vi "4Pi Dual DM - Mode Scan Engine.vi"() -> ()   [LabVIEW 2021]
uses:
  4Pi Dual DM - Controls/4Pi Dual DM - Mode Scan - Gaussian Initial Guesses.ctl
  4Pi Dual DM - Controls/4Pi Dual DM - Mode Scan - Metric Fit Type.ctl
  4Pi Dual DM - Controls/4Pi Dual DM - Mode Scan - Scan Settings.ctl
  4Pi Dual DM - Controls/4Pi Dual DM - Mode Scan - Metric.ctl
  4Pi Dual DM - Controls/4Pi Dual DM - Mode Scan - Threshold Mean Limits.ctl
  4Pi Dual DM - Controls/4Pi Dual DM - Mode Scan - Image Type.ctl
  4Pi Dual DM - Controls/4Pi Dual DM - Mode Scan - Blink Scan Settings.ctl
  4Pi Dual DM - Controls/4Pi Dual DM - Mode Scan - Blink Analysis Type.ctl
  <vilib>/vision/Image Controls.llb/IMAQ Image.ctl
  Hardware Configuration/Hardware Configuration Controls/Device Type.ctl
  Hardware Configuration/Hardware Configuration Controls/Device Function.ctl
  <vilib>/Utility/miscctls.llb/LVPointTypeDef.ctl
  4Pi Dual DM - Controls/4Pi Dual DM - Mode Scan - Last Used Data Type.ctl
  4Pi Dual DM - Controls/4Pi Dual DM - Mode Scan - Notifier Type.ctl
  4Pi Dual DM - Controls/4Pi Dual DM - Mode Scan - Scan Actions.ctl
  4Pi Dual DM - Controls/4Pi Dual DM - Standard Action.ctl
  4Pi Dual DM - Controls/4Pi Dual DM - Standard Counter Action.ctl
  <vilib>/Analysis/6fits.llb/Curve Fitting Criteria.ctl
  <vilib>/Analysis/baseanly.llb/Mean (DBL).vi
  <vilib>/Analysis/NI_AALBase.lvlib
  <vilib>/Analysis/NI_AALPro.lvlib
  <vilib>/gmath/NI_Gmath.lvlib
  <resource>/objmgr/IMAQImage.rc
panel:
  in  "Calling VI Ref":refnum<vi>
  in  "Main Tab":enum32{"Scan Modes", "Settings"}(tab)
  in  "Fit Data":bool
  in  "Apply":bool
  in  "Get Image":bool
  in  "Current Mode":i32(ring) items=["1", "2", "3", "4", "5", "6", "7", "8", "9", "10", "11", "12", "13", "14", "15", "16", "17", "18", "19", "20", "21", "22", "23", "24", "25", "26", "27", "28", "29", "30", "31", "32", "33", "34", "35", "36", "37", "38", "39", "40", "41", "42", "43", "44", "45", "46", "47", "48", "49", "50", "51", "52", "53", "54", "55", "56", "57", "58", "59", "60", "61", "62", "63", "64", "65", "66", "67", "68", "69", "70", "71", "72", "73", "74", "75", "76", "77", "78", "79", "80", "81", "82", "83", "84", "85", "86", "87", "88", "89", "90", "91", "92", "93", "94", "95", "96", "97", "98", "99", "100", "101", "102", "103", "104", "105", "106", "107", "108", "109", "110", "111", "112", "113", "114", "115", "116", "117", "118", "119", "120", "121", "122", "123", "124", "125", "126", "127", "128", "129", "130", "131", "132", "133", "134", "135", "136", "137", "138", "139", "140"]
  in  "Scan Mode":bool
  in  "Scan Next Mode":bool
  in  "Auto Scan Modes":bool
  out "Metric":cluster{dbl[], dbl[]}[](graph)
  out "AO Image Display":T1(plugin-control)
  in  "Gaussian Initial Guesses":T2={"Amplitude"=2500.0, "Center Position"=0.0, "Width (Sigma)"=200.0, "Offset"=500.0, "User Guesses"=TRUE}
  in  "DM Scan Settings":T3={"Frame Delay"=1, "Frame Accumulations"=2, "Number of Steps"=8, "Step Size (nm)"=0.5} {"Step Size (nm)" format="%.2f"}
  in  "Image Type":T4 items=["Full Image", "ROI", "Blinks"]
  in  "Image Selection":i32(ring) items=["Quad 01", "Quad 02", "Quad 03", "Quad 04"]
  in  "Metric":T5=1 items=["Max Intensity", "No Zero Mean", "Threshold Mean", "Mean"]
  in  "Metric Fit Type":T6 items=["Guassian", "Quadratic"]
  in  "Threshold Mean Limits":T7={"Upper Limit"=10000.0, "Lower Limit"=0.0}
  in  "Blink Scan Settings":T8={"Blink Analysis Type"=1, "Blink ROI Box Width"=0, "Blink Threshold"=0.0} {"Blink Analysis Type" items=["Mean Intensity", "2D Fit Intensity"]}
  in  "Exit":bool
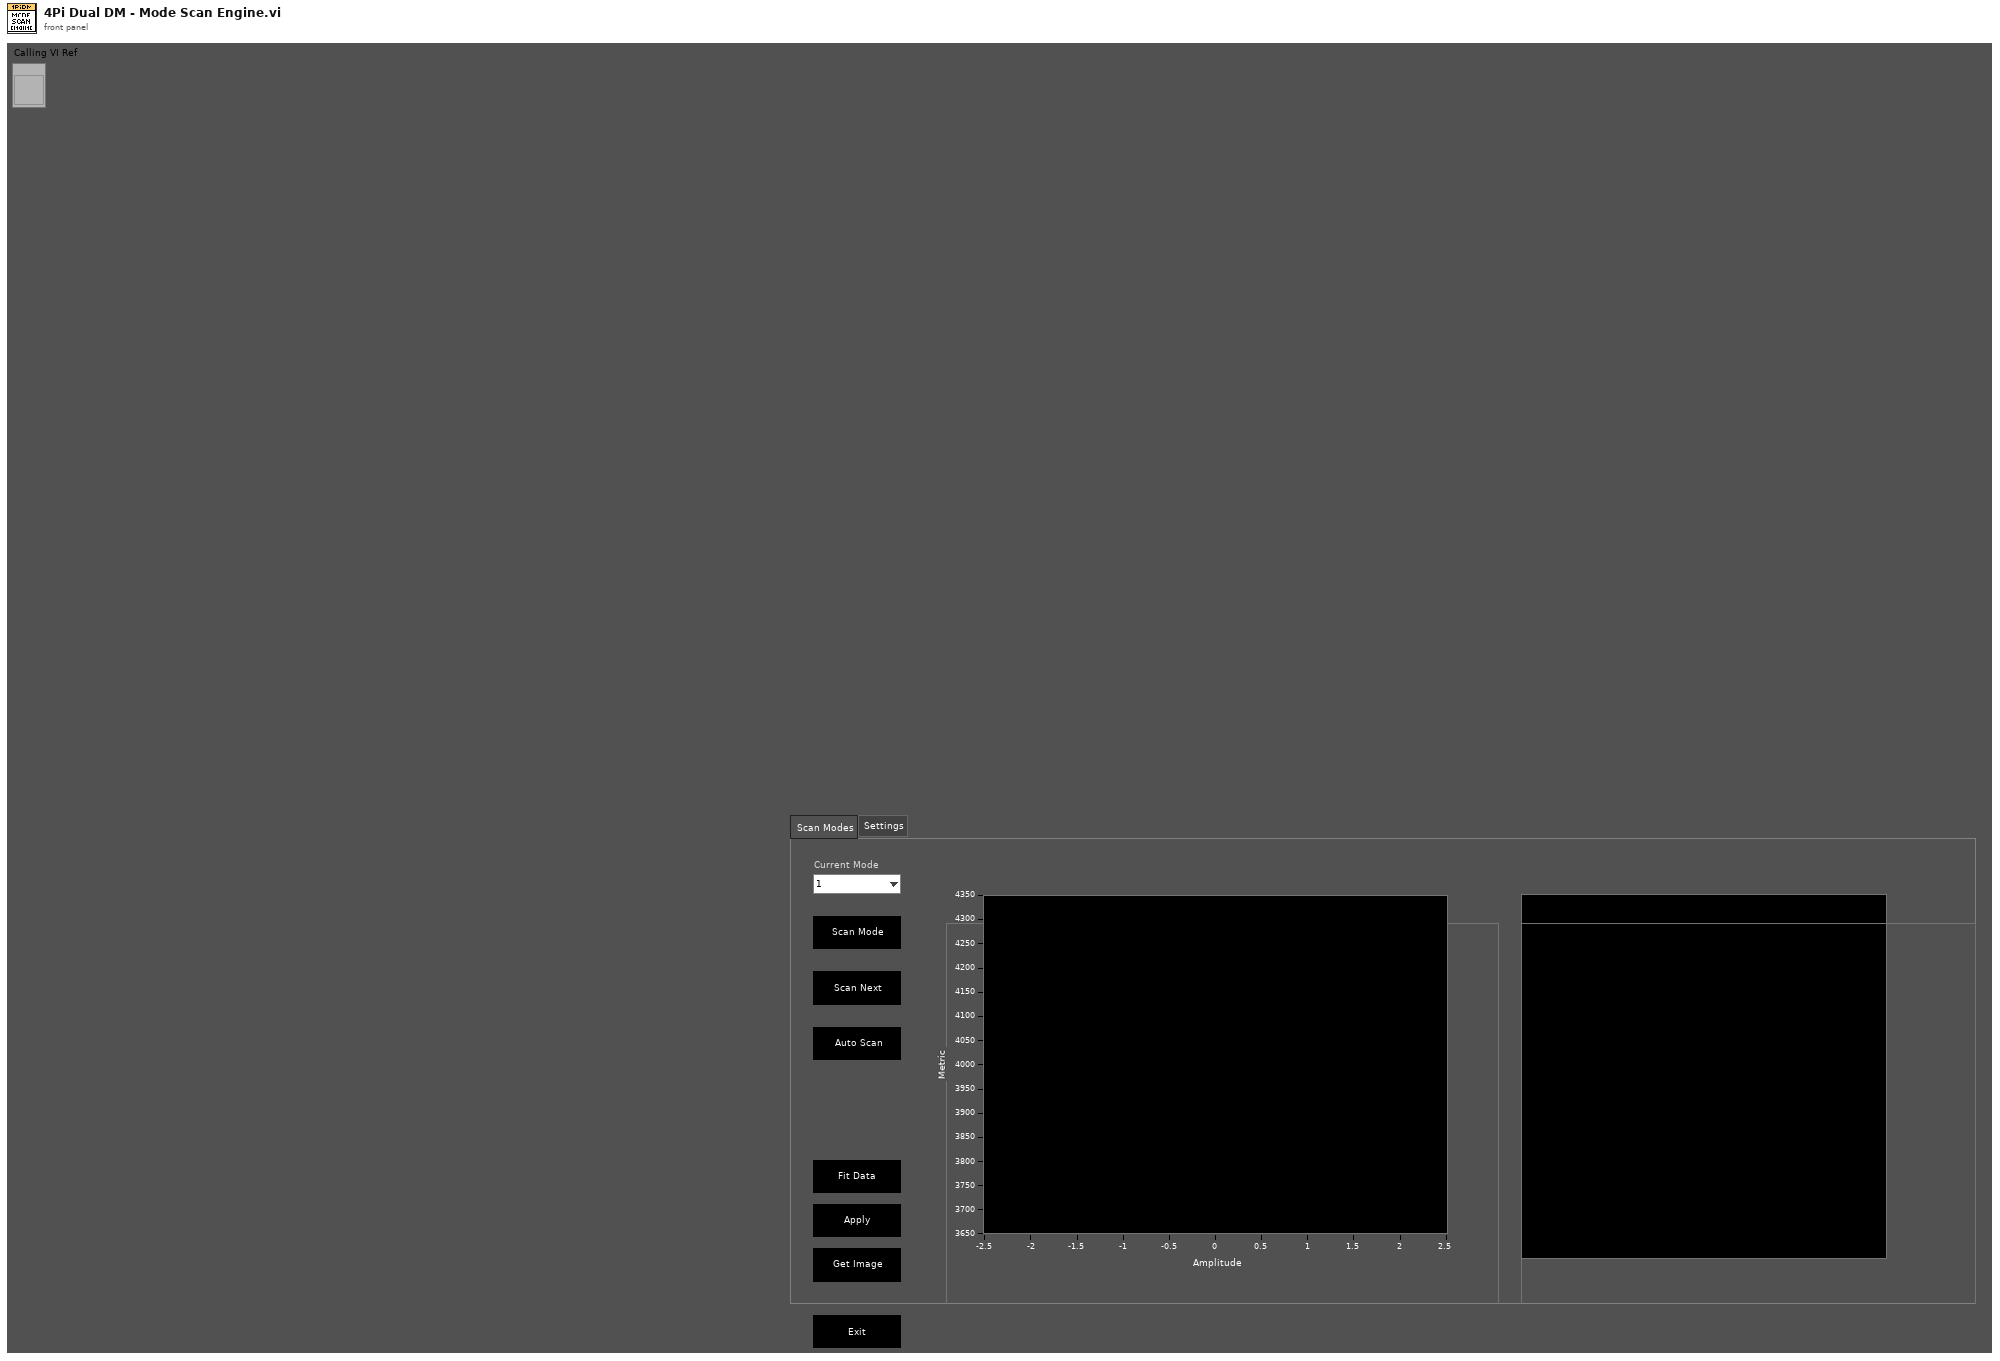
[diagram p1: front panel]
types:
  T1 = typedef "IMAQ Image.ctl" = refnum<image>
  T2 = typedef "4Pi Dual DM - Mode Scan - Gaussian Initial Guesses.ctl" = cluster{"Amplitude":dbl, "Center Position":dbl, "Width (Sigma)":dbl, "Offset":dbl, "User Guesses":bool}
  T3 = typedef "4Pi Dual DM - Mode Scan - Scan Settings.ctl" = cluster{"Frame Delay":u32, "Frame Accumulations":u16, "Number of Steps":u16, "Step Size (nm)":dbl}
  T4 = typedef "4Pi Dual DM - Mode Scan - Image Type.ctl" = u16
  T5 = typedef "4Pi Dual DM - Mode Scan - Metric.ctl" = u16
  T6 = typedef "4Pi Dual DM - Mode Scan - Metric Fit Type.ctl" = u16
  T7 = typedef "4Pi Dual DM - Mode Scan - Threshold Mean Limits.ctl" = cluster{"Upper Limit":dbl, "Lower Limit":dbl}
  T8 = typedef "4Pi Dual DM - Mode Scan - Blink Scan Settings.ctl" = cluster{"Blink Analysis Type":T9, "Blink ROI Box Width":u8, "Blink Threshold":sgl}
  T9 = typedef "4Pi Dual DM - Mode Scan - Blink Analysis Type.ctl" = u16
  T10 = typedef "Image Type" = u32
  T11 = enum8{"Enabled", "Disabled", "Disabled and Grayed Out"}
  T12 = typedef "4Pi Dual DM - Mode Scan - Scan Actions.ctl" = enum16{"Scan Mode", "Fit Data", "Scan Next Mode", "Update Mode Amount", "Get Image", "Compute Metric", "Update Counter", "Apply Correction", "Exit", "Quit"}
  T13 = typedef "4Pi Dual DM - Mode Scan - Notifier Type.ctl" = cluster{"Action":T12, "Image Ref":T1, "Image Type":T4, "Fit Type":T6, "Metric":T5, "Scan Running?":bool, "DM Scan Settings":T3, "Threshold Mean Limits":T7, "Gaussian Initial Guesses":T2, "Blink Scan Settings":T8}
  T14 = typedef "4Pi Dual DM - Mode Scan - Last Used Data Type.ctl" = cluster{"Image Ref Index":i32, "Image Type":T4, "Fit Type":T6, "Metric":T5, "DM Scan Settings":T3, "Threshold Mean Limits":T7, "Gaussian Initial Guesses":T2, "Blink Scan Settings":T8}
  T15 = enum16{"Always On", "Always Off", "Off While Running"}
  T16 = typedef "LVPointTypeDef.ctl" = cluster{"Horizontal":i16, "Vertical":i16}
  T17 = typedef "Device Function.ctl" = enum16{"Primary", "Secondary", "Overview", "Wide Field Drift Correction", "642 nm Excitation", "560 nm Excitation", "940 nm Excitation", "546 nm Excitation", "488 nm Excitation", "405 nm Excitation", "Objective Drift Correction", "4Pi Focus Lock", "4Pi Objective Lock", "Objective XY", "Objective Z", "Sample XY", "Sample Coarse Z", "Sample Z", "4Pi Lower", "4Pi Upper", "Em Small", "Em Large", "Ex Small", "Ex Large", "Mojo", "Adj Cavity", "Line Scanning", "Alert"}
  T18 = typedef "Device Type.ctl" = enum16{"AOTF", "Camera", "Deformable Mirror", "Laser", "Flip Mirror", "Shutter", "Stage", "Waveform", "FPGA", "Email"}
  T19 = typedef "LVRectTypeDef.ctl" = cluster{"Left":i16, "Top":i16, "Right":i16, "Bottom":i16}
  T20 = typedef "LVBoundsTypeDef.ctl" = cluster{"Width":u32, "Height":u32}
  T21 = typedef "4Pi Dual DM - Standard Action.ctl" = enum16{"Read", "Write"}
  T22 = typedef "4Pi Dual DM - Standard Counter Action.ctl" = enum16{"Initialize", "Update Count", "Get Count"}
  T23 = cluster{"initial amplitude":dbl, "initial center":dbl, "initial standard deviation":dbl, "offset":dbl}
  T24 = cluster{"amp min":dbl, "amp max":dbl, "center min":dbl, "center max":dbl, "deviation min":dbl, "deviation max":dbl, "offset min":dbl, "offset max":dbl}
  T25 = enum16{"Linear", "Polynomial", "Exponential", "Power"}
  T26 = typedef "4Pi Dual DM - Mirror Modes DUAL.ctl" = cluster{"Mode":string, "Amplitude":dbl}[][]
  T27 = cluster{"Global Rectangle":i32[], "Contours":cluster{"Contour Type":u32, "ROI Type":u32, "Points":i32[]}[]}
  T28 = cluster{"Amplitude Out":dbl[], "Metric Out":dbl[]}
  T29 = cluster{"initial amplitude":dbl, "Numeric":dbl, "initial standard deviation":dbl, "offset":dbl}
  T30 = typedef "NI_AALPro.lvlib/Curve Fitting Criteria.ctl" = u16
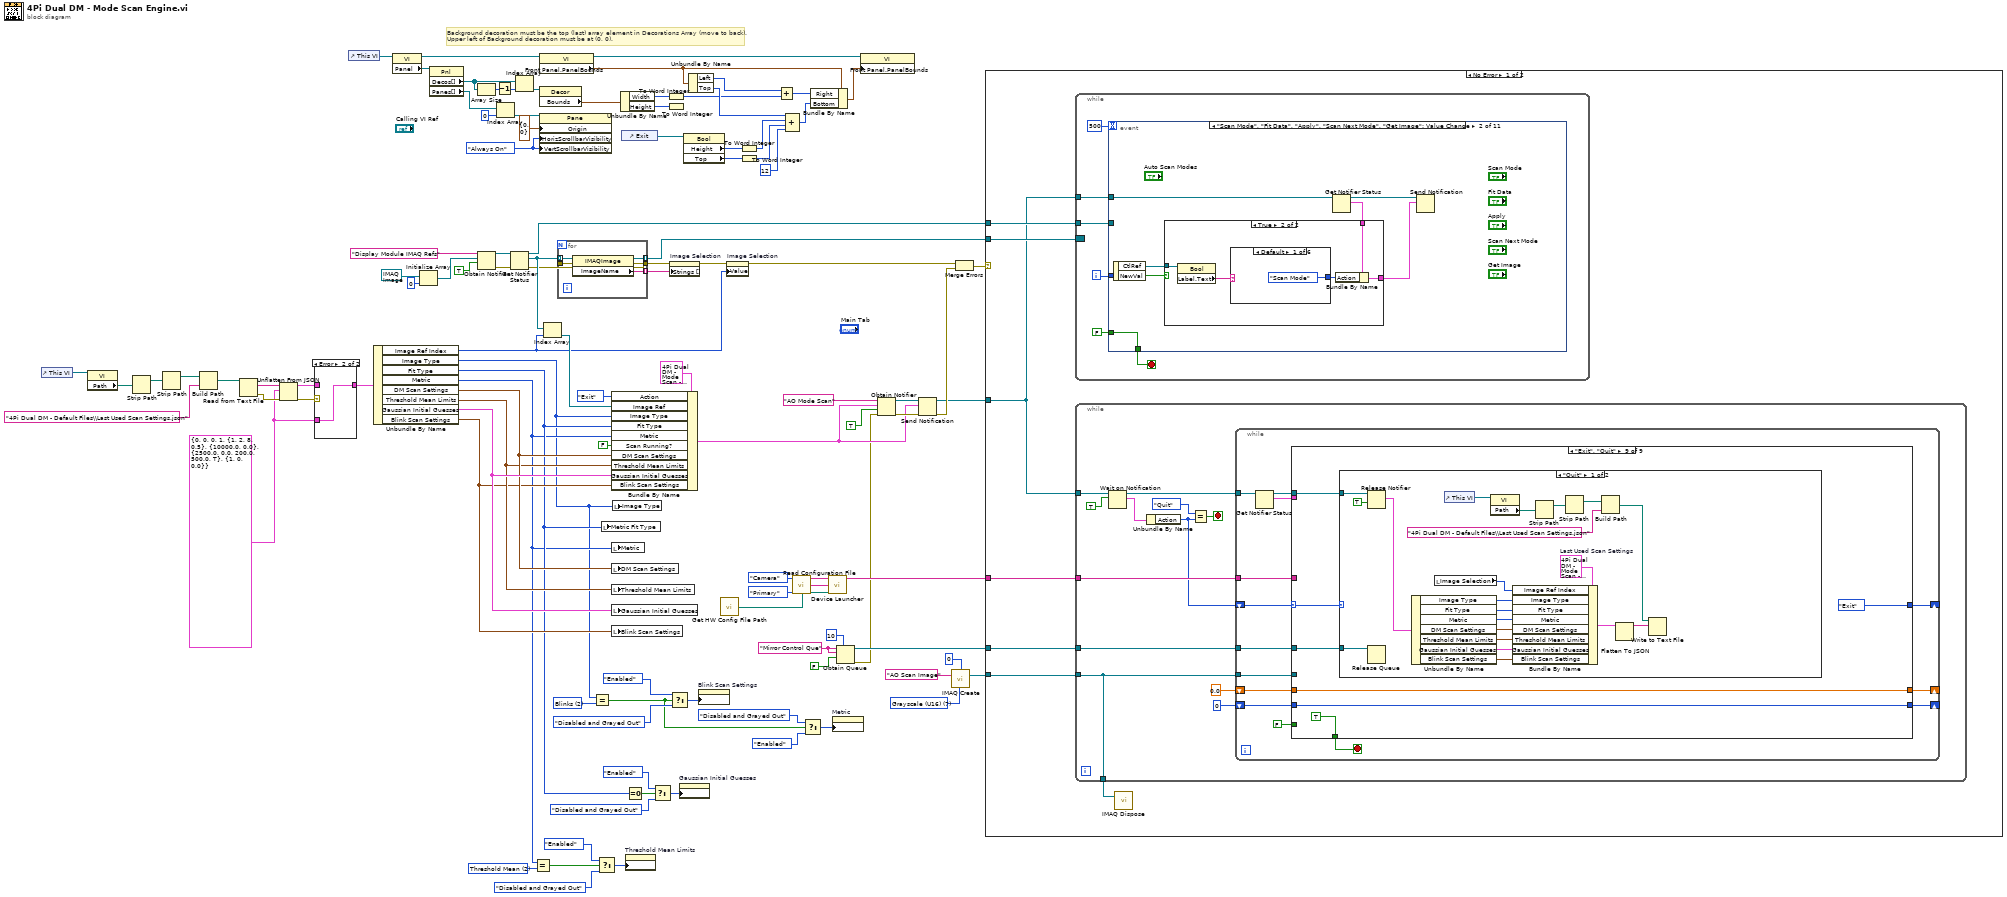
[diagram p0: block diagram]
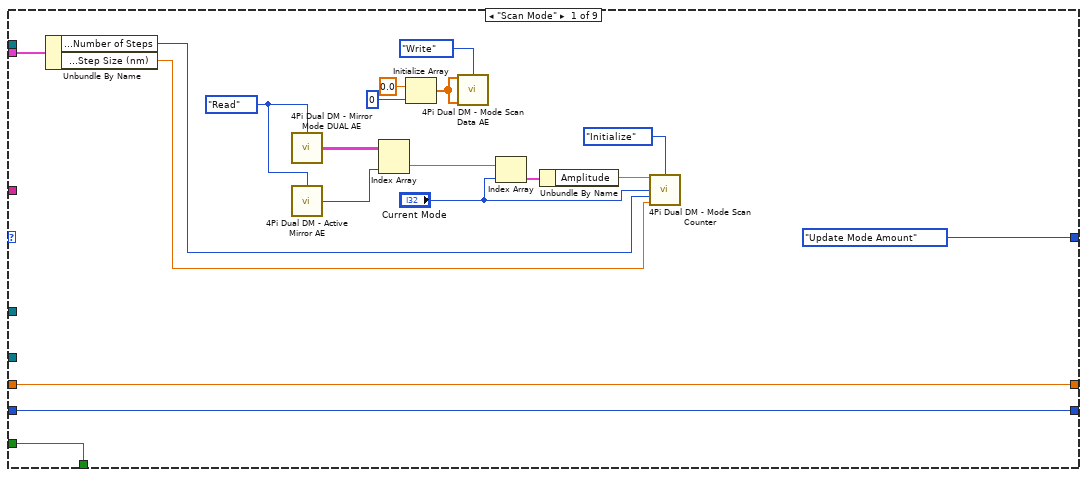
[diagram p2: hidden frame]
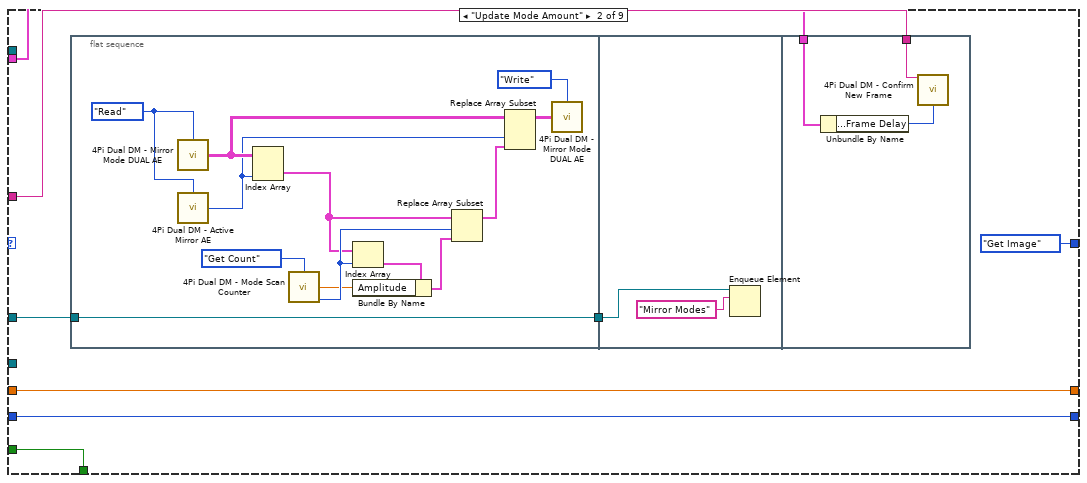
[diagram p3: hidden frame]
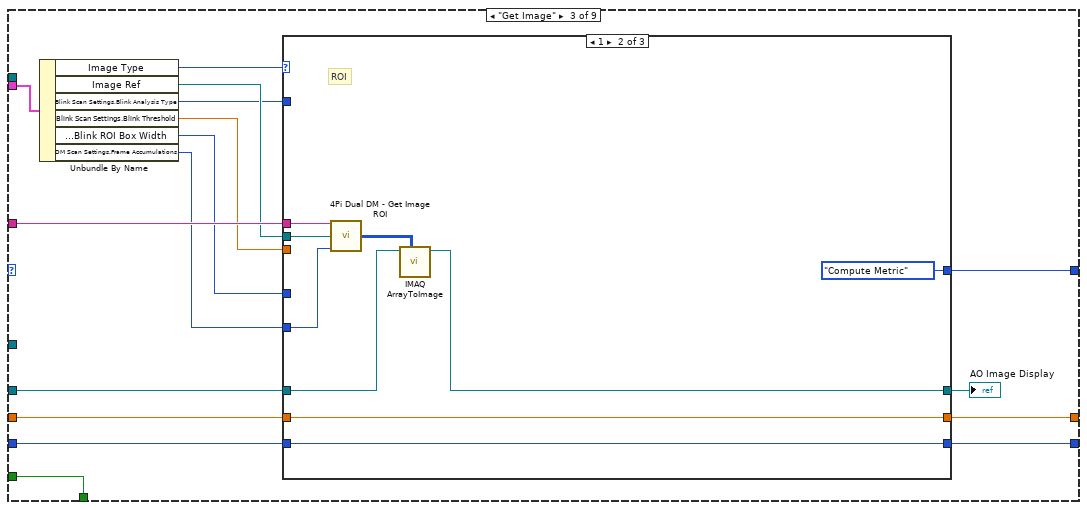
[diagram p4: hidden frame]
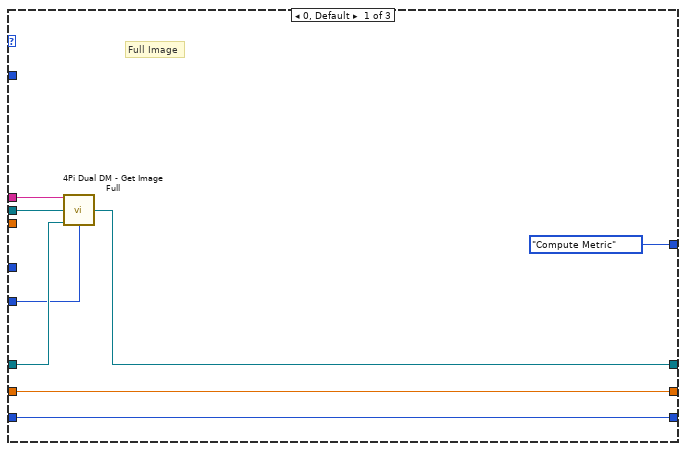
[diagram p5: hidden frame]
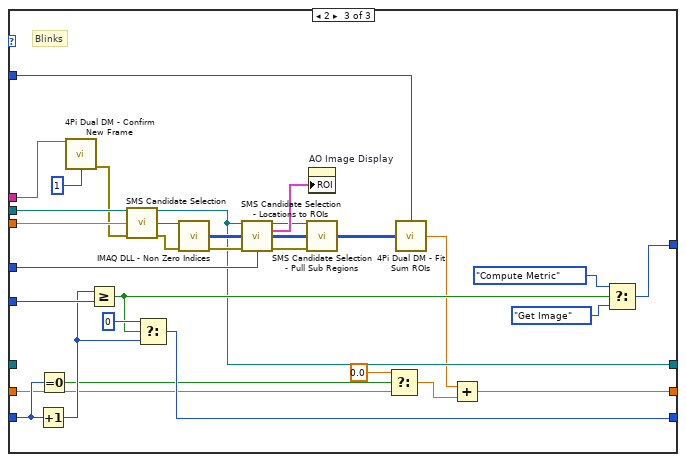
[diagram p6: hidden frame]
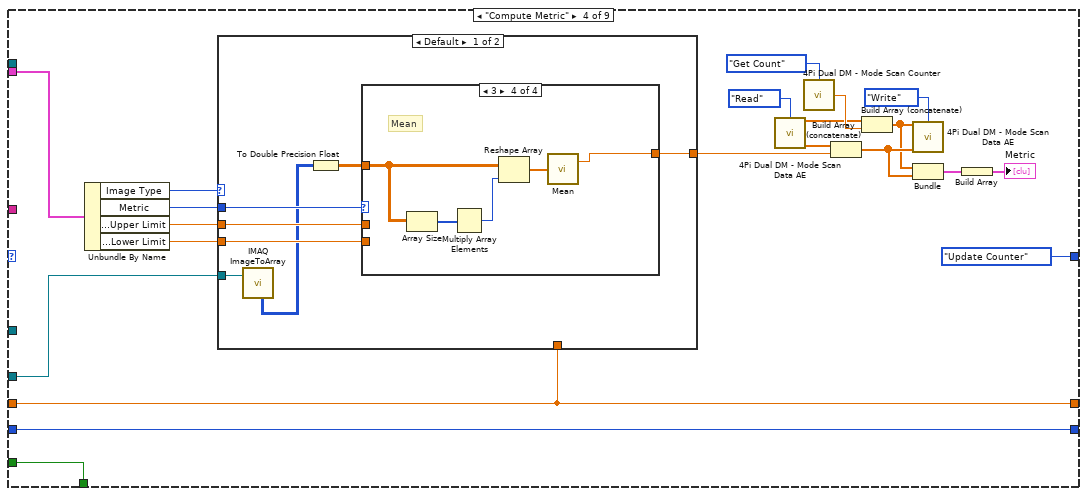
[diagram p7: hidden frame]
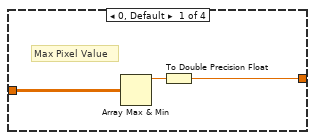
[diagram p8: hidden frame]
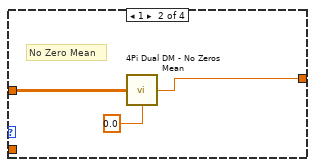
[diagram p9: hidden frame]
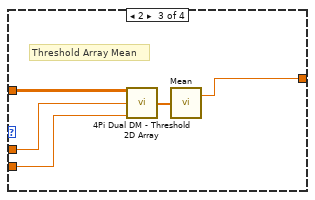
[diagram p10: hidden frame]
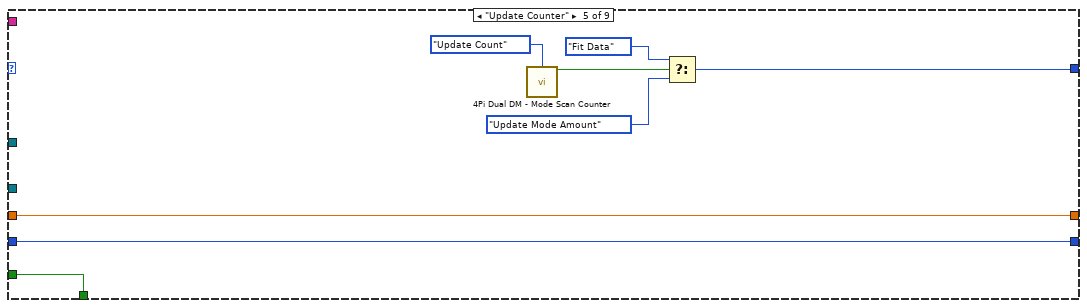
[diagram p12: hidden frame]
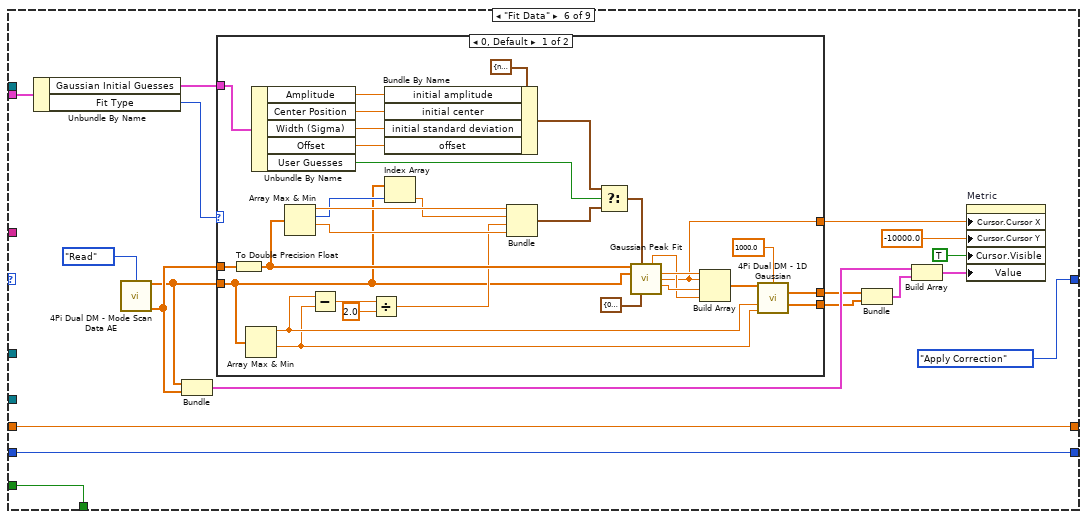
[diagram p13: hidden frame]
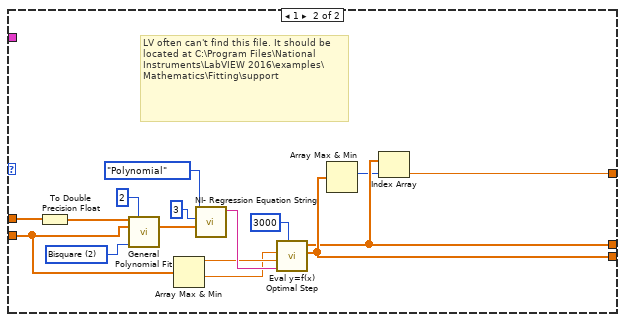
[diagram p14: hidden frame]
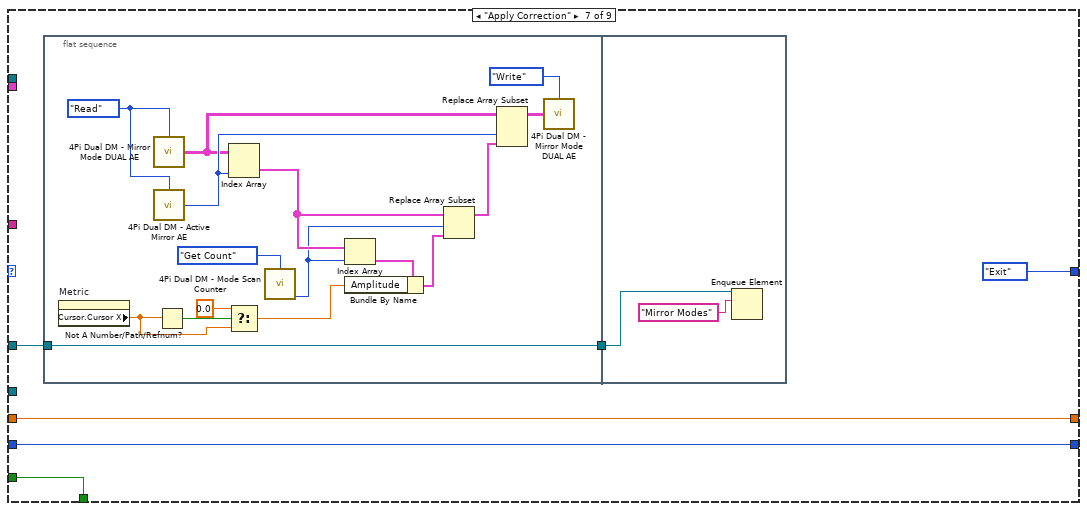
[diagram p15: hidden frame]
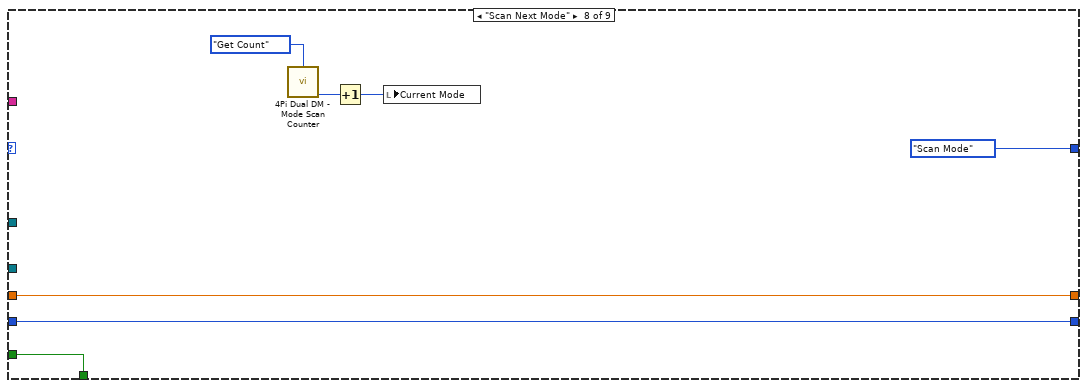
[diagram p16: hidden frame]
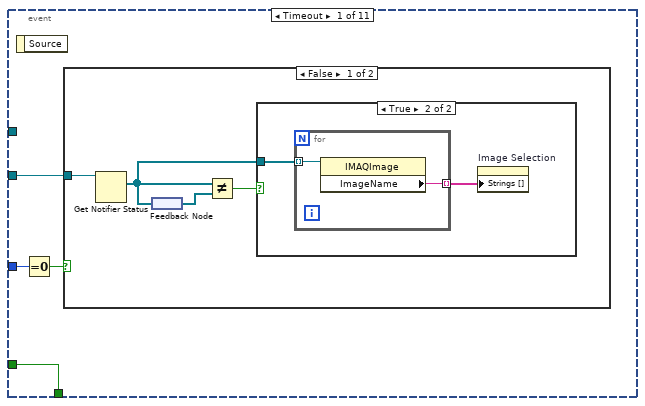
[diagram p18: hidden frame]
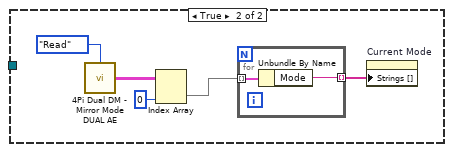
[diagram p20: hidden frame]
diagram:
  w2 = T10 7 items=["Grayscale (U8)", "Grayscale (I16)", "Grayscale (SGL)", "Complex (CSG)", "RGB (U32)", "HSL (U32)", "RGB (U64)", "Grayscale (U16)"] ("Image Type")
  w12 = T4 2 items=["Full Image", "ROI", "Blinks"] ("y")
  w15 = T5 2 items=["Max Intensity", "No Zero Mean", "Threshold Mean", "Mean"] ("y")
  w45 = T14 {"Image Ref Index"=0, "Image Type"=0, "Fit Type"=0, "Metric"=1, "DM Scan Settings"={"Frame Delay"=1, "Frame Accumulations"=2, "Number of Steps"=8, "Step Size (nm)"=0.5}, "Threshold Mean Limits"={"Upper Limit"=10000.0, "Lower Limit"=0.0}, "Gaussian Initial Guesses"={"Amplitude"=2500.0, "Center Position"=0.0, "Width (Sigma)"=200.0, "Offset"=500.0, "User Guesses"=TRUE}, "Blink Scan Settings"={"Blink Analysis Type"=1, "Blink ROI Box Width"=0, "Blink Threshold"=0.0}} ("Mode Scan Notifier Type")
  w76 = T15."Always On" ("Vertical Scrollbar Visibility")
  w109 = "Mirror Control Que" ("name (unnamed)")
  # "Background decoration must be the top (last) array element in Decorations Array (move to back).\nUpper left of Background decoration must be at (0, 0)."
  n1 = control-ref of="This VI"() -> (w58:refnum<vi>)
  n2 = property class="VI"(reference=w58) -> ("Path"=w57:path)  [unwired: 1 in, 2 out]
  n3 = Strip Path(path=w57) -> (stripped path=w56:path)  [unwired: 1 out]
  n4 = Strip Path(path=w56) -> (stripped path=w55:path)  [unwired: 1 out]
  n5 = Build Path(base path=w55, name or relative path="4Pi Dual DM - Default Files\\Last Used Scan Settings.json") -> (appended path=w52:path)
  n6 = Read from Text File(file (use dialog)=w52) -> (text=w53:string, error out=w51:errorcluster)  [unwired: 3 in, 2 out]
  n7 = Unflatten From JSON(JSON string=w53, type and defaults=w45, error in (no error)=w51) -> (value=w44:T14, error out=w50:errorcluster)  [unwired: 4 in]
  n8 = case shown="Error" w50 {
    tunnel: w45 -> [_ w111]
    tunnel: w44 -> [w110 _]
    tunnel: [w110 w111] -> w41
    frame No Error {
    }
    frame Error {
    }
  }
  n9 = control-ref of="This VI"() -> (w68:refnum<vi>)
  n10 = Unbundle By Name(w41) -> ("Image Ref Index"=w39:i32, "Image Type"=w9:T4, "Fit Type"=w24:T6, "Metric"=w14:T5, "DM Scan Settings"=w27:T3, "Threshold Mean Limits"=w26:T7, "Gaussian Initial Guesses"=w28:T2, "Blink Scan Settings"=w25:T8)
  n11 = property class="VI"(reference=w68) -> (reference out=w77:refnum<vi>, "Panel"=w69:refnum<vi>)  [unwired: 1 in, 1 out]
  n12 = Initialize Array(T1 refnum ("New Image"), 0 ("dimension size")) -> (w102:T1[])
  n13 = property class="Pnl"(reference=w69) -> ("Decos[]"=w67:refnum<vi>[], "Panes[]"=w73:refnum<vi>[])  [unwired: 1 in, 2 out]
  n14 = Obtain Notifier(name (unnamed)="Display Module IMAQ Refs", notification data type=w102, create if not found? (T)=TRUE) -> (notifier out=w101:refnum<notifier>, error out=w63:errorcluster)  [unwired: 1 in, 1 out]
  n15 = Array Size(array=w67) -> (size(s)=w65:i32)
  n16 = Decrement(x=w65) -> (x-1=w66:i32)
  n17 = Index Array(array=w73, index=0) -> (element=w72:refnum<vi>)
  n18 = Get Notifier Status(notifier=w101, error in (no error)=w63) -> (notifier out=w34:refnum<notifier>, current notification=w64:T1[], error out=w62:errorcluster)  [unwired: 2 out]
  n19 = Index Array(array=w67, index=w66) -> (element=w75:refnum<vi>)
  n20 = Equal?(x=w14, y=w15) -> (x = y?=w16:bool)
  n21 = property class="VI"(reference=w77) -> (reference out=w79:refnum<vi>, "Front Panel.PanelBounds"=w80:T19)  [unwired: 1 in, 1 out]
  n22 = property class="Decor"(reference=w75) -> ("Bounds"=w78:T20)  [unwired: 1 in, 2 out]
  n23 = property class="Pane"(reference=w72, "Origin"=T16 {"Horizontal"=0, "Vertical"=0}, "HorizScrollbarVisibility"=w76, "VertScrollbarVisibility"=w76) -> ()  [unwired: 1 in, 2 out]
  n24 = Index Array(array=w64, index=w39) -> (element=w40:T1)
  n25 = for {
    tunnel: w64 -> [w116] mode=indexing
    tunnel: [w115] -> w61 mode=indexing
    tunnel: [w114] -> w60
    tunnel: [w113] -> w33 mode=indexing
    tunnel: w62 -> [w112]
    n26 = property class="IMAQImage"(reference=w116, error in=w112) -> (reference out=w113:T1, error out=w114:errorcluster, "ImageName"=w115:string)
  }
  n27 = Equal?(x=w9, y=w12) -> (x = y?=w5:bool)
  n28 = Select(t=T11."Enabled" ("Disabled"), s=w16, f=T11."Disabled and Grayed Out" ("Disabled")) -> (s? t:f=w19:T11)
  n29 = local write "Metric Fit Type"(w24) -> ()
  n30 = Bundle By Name(cluster=T13 {"Action"=enum."Scan Mode", "Image Ref"=refnum, "Image Type"=0, "Fit Type"=0, "Metric"=1, "Scan Running?"=FALSE, "DM Scan Settings"={"Frame Delay"=1, "Frame Accumulations"=2, "Number of Steps"=8, "Step Size (nm)"=80.0}, "Threshold Mean Limits"={"Upper Limit"=10000.0, "Lower Limit"=0.0}, "Gaussian Initial Guesses"={"Amplitude"=2500.0, "Center Position"=0.0, "Width (Sigma)"=200.0, "Offset"=500.0, "User Guesses"=TRUE}, "Blink Scan Settings"={"Blink Analysis Type"=1, "Blink ROI Box Width"=0, "Blink Threshold"=0.0}} ("Mode Scan Notifier Type"), "Action"=4Pi_Dual_DM_-_Mode_Scan_-_Scan_Actions."Exit", "Image Ref"=w40, "Image Type"=w9, "Fit Type"=w24, "Metric"=w14, "Scan Running?"=FALSE, "DM Scan Settings"=w27, "Threshold Mean Limits"=w26, "Gaussian Initial Guesses"=w28, "Blink Scan Settings"=w25) -> (w37:T13)
  n31 = local write "Metric"(w14) -> ()
  n32 = local write "DM Scan Settings"(w27) -> ()
  n33 = local write "Threshold Mean Limits"(w26) -> ()
  n34 = local write "Gaussian Initial Guesses"(w28) -> ()
  n35 = local write "Blink Scan Settings"(w25) -> ()
  n36 = local write "Image Type"(w9) -> ()
  n37 = Unbundle By Name(w78) -> ("Width"=w83:u32, "Height"=w86:u32)
  n38 = control-ref of="Exit"() -> (w70:refnum<vi>)
  n39 = property on="Threshold Mean Limits" class="Clust (strict)"("DisabledEnum"=w19) -> ()  [unwired: 2 in, 2 out]
  n40 = Equal To 0?(x=w24) -> (x = 0?=w23:bool)
  n41 = Select(t=T11."Enabled" ("Disabled"), s=w23, f=T11."Disabled and Grayed Out" ("Disabled")) -> (s? t:f=w20:T11)
  n42 = To Word Integer(number=w83) -> (16bit integer=w85:i16)
  n43 = To Word Integer(number=w86) -> ()  [unwired: 1 out]
  n44 = property on="Image Selection" class="Ring (strict)"(error in=w60, "Strings []"=w61) -> (error out=w59:errorcluster)  [unwired: 1 in, 1 out]
  n45 = Select(t=T11."Enabled" ("Disabled"), s=w5, f=T11."Disabled and Grayed Out" ("Disabled")) -> (s? t:f=w13:T11)
  n46 = property on="Gaussian Initial Guesses" class="Clust (strict)"("DisabledEnum"=w20) -> ()  [unwired: 2 in, 2 out]
  n47 = property class="Bool"(reference=w70) -> ("Height"=w88:u32, "Top"=w89:i32)  [unwired: 1 in, 2 out]
  n48 = Unbundle By Name(w80) -> ("Left"=w82:i16, "Top"=w93:i16)
  n49 = property on="Blink Scan Settings" class="Clust (strict)"("DisabledEnum"=w13) -> ()  [unwired: 2 in, 2 out]
  n50 = call "Get HW Config File Path.vi"() -> ("File Path"=w95:path)  [unwired: 14 in, 1 out]
  n51 = property on="Image Selection" class="Ring (strict)"(error in=w59, "Value"=w39) -> (error out=w32:errorcluster)  [unwired: 1 in, 1 out]
  n52 = To Word Integer(number=w88) -> (16bit integer=w91:i16)
  n53 = To Word Integer(number=w89) -> (16bit integer=w92:i16)
  n54 = Add(x=w82, y=w85) -> (x+y=w84:i16)
  n55 = Compound Arithmetic op=ADD(w93, w91, w92, i16 12 ("y")) -> (w87:i16)
  n56 = call "Read Configuration File.vi"("Device Type"=Device_Type."Camera", "Device Function"=Device_Function."Primary", "Config File Path"=w95) -> ("Unique Notifier Name"=w96:string, "Device Ports/IDs/Channels"=w98:string[], "Device Engine Path"=w97:path)  [unwired: 9 in, 1 out]
  n57 = Select(t=T11."Disabled and Grayed Out" ("Disabled"), s=w5, f=T11."Enabled" ("Disabled")) -> (s? t:f=w6:T11)
  n58 = Bundle By Name(cluster=w80, "Right"=w84, "Bottom"=w87) -> (w81:T19)
  n59 = call "Device Launcher.vi"("Notifier Name"=w96, "Device Ports/IDs/Channels"=w98, "Device Engine Path"=w97) -> ("Notifier Name"=w94:string)  [unwired: 11 in, 1 out]
  n60 = property on="Metric" class="Ring (strict)"("DisabledEnum"=w6) -> ()  [unwired: 2 in, 2 out]
  n61 = Obtain Queue(max queue size (-1, unlimited)=10, name (unnamed)=w109, element data type=w109, create if not found? (T)=FALSE) -> (queue out=w107:refnum<queue>, error out=w35:errorcluster)  [unwired: 1 in, 1 out]
  n62 = property class="VI"(reference=w79, "Front Panel.PanelBounds"=w81) -> ()  [unwired: 1 in, 2 out]
  n63 = Obtain Notifier(name (unnamed)="AO Mode Scan", notification data type=w37, create if not found? (T)=TRUE, error in (no error)=w35) -> (notifier out=w46:refnum<notifier>, error out=w47:errorcluster)  [unwired: 1 out]
  n64 = Send Notification(notification=w37, notifier=w46, error in (no error)=w47) -> (notifier out=w29:refnum<notifier>, error out=w31:errorcluster)
  n65 = call "IMAQ Create"("Border Size"=0, "Image Name"="AO Scan Image", "Image Type"=w2) -> ("New Image"=w1:T1)  [unwired: 2 in, 1 out]
  n66 = Merge Errors(w32, w31) -> (w30:errorcluster)
  n67 = case shown="No Error" w30 {
    tunnel: w107 -> [w123 w567]
    tunnel: w94 -> [w122 _]
    tunnel: w34 -> [w121 w565]
    tunnel: w33 -> [w120 _]
    tunnel: w29 -> [w119 w566]
    tunnel: w1 -> [w118 w568]
    frame No Error {
      n68 = while {
        tunnel: w121 -> [w440]
        border: w120 -> [_]
        tunnel: w119 -> [w439]
        i -> [w442]
        stop <- w437 stop-if-true
        n69 = event shown="[1] \"Scan Mode\", \"Fit Data\", \"Apply\", \"Scan Next Mode\", \"Get Image\": Value Change" {
          selector: _ -> [_ _ _ _ _ _ _ _ _ _ _]
          dyn-events: _ -> [_ _ _ _ _ _ _ _ _ _ _]
          timeout: 500 -> [_ _ _ _ _ _ _ _ _ _ _]
          tunnel: w442 -> [w446 _ _ _ _ _ _ _ _ _ _]
          tunnel: w440 -> [w444 _ w492 _ _ _ _ _ _ _ w564]
          tunnel: w439 -> [_ w467 w491 w500 w513 w528 w536 w543 w550 w557 w562]
          tunnel: [w443 w463 w483 w493 w514 w529 w530 w537 w544 w551 TRUE] -> w437
          tunnel: FALSE -> [w443 w463 w483 w493 w514 w529 w530 w537 w544 w551 _]
          event Timeout {
            n70 = event-data() -> ()  [unwired: 1 in, 1 out]
            n71 = Equal To 0?(x=w446) -> (x = 0?=w445:bool)
            n72 = case shown="False" w445 {
              tunnel: w444 -> [w450 _]
              frame False {
                n73 = Get Notifier Status(notifier=w450) -> (current notification=w447:T1[])  [unwired: 1 in, 4 out]
                n74 = feedback-in #1(w447) -> ()
                n75 = feedback #1() -> (w449:T1[])
                n76 = Not Equal?(x=w447, y=w449) -> (x != y?=w448:bool)
                n77 = case shown="True" w448 {
                  tunnel: w447 -> [_ w452]
                  frame False {
                  }
                  frame True {
                    n78 = for {
                      tunnel: w452 -> [w454] mode=indexing
                      tunnel: [w453] -> w451 mode=indexing
                      n79 = property class="IMAQImage"(reference=w454) -> ("ImageName"=w453:string)  [unwired: 1 in, 2 out]
                    }
                    n80 = property on="Image Selection" class="Ring (strict)"("Strings []"=w451) -> ()  [unwired: 2 in, 2 out]
                  }
                }
              }
              frame True {
                n81 = call "4Pi Dual DM - Mirror Mode DUAL AE.vi"("Action"=4Pi_Dual_DM_-_Standard_Action."Read") -> ("Mirror Modes Out"=w457:T26)  [unwired: 14 in]
                n82 = Index Array(array=w457, index (col)=0 ("disabled index (col)")) -> (element=w455:cluster{"Mode":string, "Amplitude":dbl}[])  [unwired: 1 in]
                n83 = for {
                  tunnel: w455 -> [w461] mode=indexing
                  tunnel: [w460] -> w459 mode=indexing
                  n84 = Unbundle By Name(w461) -> ("Mode"=w460:string)
                }
                n85 = property on="Current Mode" class="Ring (strict)"("Strings []"=w459) -> ()  [unwired: 2 in, 2 out]
              }
            }
          }
          event "Scan Mode", "Fit Data", "Apply", "Scan Next Mode", "Get Image": Value Change {
            n86 = event-data() -> ("CtlRef"=w468:refnum<vi>, "NewVal"=w462:bool)  [unwired: 1 in]
            n87 = Get Notifier Status(notifier=w467) -> (notifier out=w466:refnum<notifier>, current notification=w465:T13)  [unwired: 1 in, 3 out]
            n88 = case shown="True" w462 {
              tunnel: w468 -> [_ w476]
              tunnel: w465 -> [w471 w475]
              tunnel: [w470 w474] -> w464
              frame False {
                n89 = Bundle By Name(cluster=w471, "Scan Running?"=FALSE) -> (w470:T13)
              }
              frame True {
                n90 = property class="Bool"(reference=w476) -> ("Label.Text"=w473:string)  [unwired: 1 in, 2 out]
                n91 = case shown="Default" w473 {
                  tunnel: [4Pi_Dual_DM_-_Mode_Scan_-_Scan_Actions."Scan Mode" ("Action") 4Pi_Dual_DM_-_Mode_Scan_-_Scan_Actions."Scan Mode" ("Action") 4Pi_Dual_DM_-_Mode_Scan_-_Scan_Actions."Fit Data" ("Action") 4Pi_Dual_DM_-_Mode_Scan_-_Scan_Actions."Apply Correction" ("Action") 4Pi_Dual_DM_-_Mode_Scan_-_Scan_Actions."Scan Next Mode" ("Action") 4Pi_Dual_DM_-_Mode_Scan_-_Scan_Actions."Get Image" ("Action")] -> w472
                  frame Default {
                  }
                  frame "Scan Mode" {
                  }
                  frame "Fit Data" {
                  }
                  frame "Apply" {
                  }
                  frame "Scan Next Mode" {
                  }
                  frame "Get Image" {
                  }
                }
                n92 = Bundle By Name(cluster=w475, "Action"=w472) -> (w474:T13)
              }
            }
            n93 = Send Notification(notification=w464, notifier=w466) -> ()  [unwired: 1 in, 2 out]
          }
          event "Image Selection": Value Change {
            n94 = event-data() -> ("NewVal"=w484:i32)  [unwired: 1 in]
            n95 = Get Notifier Status(notifier=w492) -> (current notification=w490:T1[])  [unwired: 1 in, 4 out]
            n96 = Index Array(array=w490, index=w484) -> (element=w488:T1)
            n97 = Get Notifier Status(notifier=w491) -> (notifier out=w486:refnum<notifier>, current notification=w489:T13)  [unwired: 1 in, 3 out]
            n98 = Bundle By Name(cluster=w489, "Image Ref"=w488, "Action"=4Pi_Dual_DM_-_Mode_Scan_-_Scan_Actions."Exit") -> (w487:T13)
            n99 = Send Notification(notification=w487, notifier=w486) -> ()  [unwired: 1 in, 2 out]
          }
          event Value Change {
            n100 = event-data() -> ("NewVal"=w495:T6)  [unwired: 1 in]
            n101 = Get Notifier Status(notifier=w500) -> (notifier out=w497:refnum<notifier>, current notification=w499:T13)  [unwired: 1 in, 3 out]
            n102 = case shown="0, Default" w495 {
              tunnel: [T11."Enabled" ("Disabled") T11."Disabled and Grayed Out" ("Disabled")] -> w494
              frame 0, Default {
              }
              frame 1 {
              }
            }
            n103 = Bundle By Name(cluster=w499, "Fit Type"=w495, "Action"=4Pi_Dual_DM_-_Mode_Scan_-_Scan_Actions."Exit") -> (w498:T13)
            n104 = Send Notification(notification=w498, notifier=w497) -> ()  [unwired: 1 in, 2 out]
            n105 = property on="Gaussian Initial Guesses" class="Clust (strict)"("DisabledEnum"=w494) -> ()  [unwired: 2 in, 2 out]
          }
          event Value Change {
            w507 = T5 2 items=["Max Intensity", "No Zero Mean", "Threshold Mean", "Mean"] ("y")
            n106 = event-data() -> ("NewVal"=w508:T5)  [unwired: 1 in]
            n107 = Equal?(x=w508, y=w507) -> (x = y?=w506:bool)
            n108 = Get Notifier Status(notifier=w513) -> (notifier out=w511:refnum<notifier>, current notification=w512:T13)  [unwired: 1 in, 3 out]
            n109 = Bundle By Name(cluster=w512, "Metric"=w508, "Action"=4Pi_Dual_DM_-_Mode_Scan_-_Scan_Actions."Exit") -> (w510:T13)
            n110 = Select(t=T11."Enabled" ("Disabled"), s=w506, f=T11."Disabled and Grayed Out" ("Disabled")) -> (s? t:f=w503:T11)
            n111 = property on="Threshold Mean Limits" class="Clust (strict)"("DisabledEnum"=w503) -> ()  [unwired: 2 in, 2 out]
            n112 = Send Notification(notification=w510, notifier=w511) -> ()  [unwired: 1 in, 2 out]
          }
          event Value Change {
            w520 = T4 2 items=["Full Image", "ROI", "Blinks"] ("y")
            n113 = event-data() -> ("NewVal"=w521:T4)  [unwired: 1 in]
            n114 = Equal?(x=w521, y=w520) -> (x = y?=w515:bool)
            n115 = Get Notifier Status(notifier=w528) -> (notifier out=w526:refnum<notifier>, current notification=w527:T13)  [unwired: 1 in, 3 out]
            n116 = Bundle By Name(cluster=w527, "Image Type"=w521, "Action"=4Pi_Dual_DM_-_Mode_Scan_-_Scan_Actions."Exit") -> (w525:T13)
            n117 = Select(t=T11."Enabled" ("Disabled"), s=w515, f=T11."Disabled and Grayed Out" ("Disabled")) -> (s? t:f=w519:T11)
            n118 = Send Notification(notification=w525, notifier=w526) -> ()  [unwired: 1 in, 2 out]
            n119 = property on="Blink Scan Settings" class="Clust (strict)"("DisabledEnum"=w519) -> ()  [unwired: 2 in, 2 out]
            n120 = Select(t=T11."Disabled and Grayed Out" ("Disabled"), s=w515, f=T11."Enabled" ("Disabled")) -> (s? t:f=w516:T11)
            n121 = property on="Metric" class="Ring (strict)"("DisabledEnum"=w516) -> ()  [unwired: 2 in, 2 out]
          }
          event Value Change {
            n122 = event-data() -> ("NewVal"=w531:T2)  [unwired: 1 in]
            n123 = Get Notifier Status(notifier=w536) -> (notifier out=w533:refnum<notifier>, current notification=w535:T13)  [unwired: 1 in, 3 out]
            n124 = Bundle By Name(cluster=w535, "Gaussian Initial Guesses"=w531, "Action"=4Pi_Dual_DM_-_Mode_Scan_-_Scan_Actions."Exit") -> (w534:T13)
            n125 = Send Notification(notification=w534, notifier=w533) -> ()  [unwired: 1 in, 2 out]
          }
          event Value Change {
            n126 = event-data() -> ("NewVal"=w538:T3)  [unwired: 1 in]
            n127 = Get Notifier Status(notifier=w543) -> (notifier out=w540:refnum<notifier>, current notification=w542:T13)  [unwired: 1 in, 3 out]
            n128 = Bundle By Name(cluster=w542, "DM Scan Settings"=w538, "Action"=4Pi_Dual_DM_-_Mode_Scan_-_Scan_Actions."Exit") -> (w541:T13)
            n129 = Send Notification(notification=w541, notifier=w540) -> ()  [unwired: 1 in, 2 out]
          }
          event Value Change {
            n130 = event-data() -> ("NewVal"=w545:T7)  [unwired: 1 in]
            n131 = Get Notifier Status(notifier=w550) -> (notifier out=w547:refnum<notifier>, current notification=w549:T13)  [unwired: 1 in, 3 out]
            n132 = Bundle By Name(cluster=w549, "Threshold Mean Limits"=w545, "Action"=4Pi_Dual_DM_-_Mode_Scan_-_Scan_Actions."Exit") -> (w548:T13)
            n133 = Send Notification(notification=w548, notifier=w547) -> ()  [unwired: 1 in, 2 out]
          }
          event Value Change {
            n134 = event-data() -> ("NewVal"=w552:T8)  [unwired: 1 in]
            n135 = Get Notifier Status(notifier=w557) -> (notifier out=w554:refnum<notifier>, current notification=w556:T13)  [unwired: 1 in, 3 out]
            n136 = Bundle By Name(cluster=w556, "Blink Scan Settings"=w552, "Action"=4Pi_Dual_DM_-_Mode_Scan_-_Scan_Actions."Exit") -> (w555:T13)
            n137 = Send Notification(notification=w555, notifier=w554) -> ()  [unwired: 1 in, 2 out]
          }
          event "Exit": Value Change {
            n138 = event-data() -> ()  [unwired: 1 in, 1 out]
            n139 = Release Notifier(notifier=w564) -> ()  [unwired: 2 in, 3 out]
            n140 = Get Notifier Status(notifier=w562) -> (notifier out=w563:refnum<notifier>, current notification=w561:T13)  [unwired: 1 in, 3 out]
            n141 = Bundle By Name(cluster=w561, "Action"=4Pi_Dual_DM_-_Mode_Scan_-_Scan_Actions."Quit") -> (w560:T13)
            n142 = Send Notification(notification=w560, notifier=w563) -> ()  [unwired: 1 in, 2 out]
          }
        }
      }
      n143 = while {
        tunnel: w123 -> [w135]
        tunnel: w122 -> [w134]
        tunnel: w119 -> [w133]
        tunnel: w118 -> [w126]
        tunnel: [w126] -> w117
        stop <- w129 stop-if-true
        n144 = Wait on Notification(notifier=w133, ignore previous (F)=TRUE) -> (notifier out=w130:refnum<notifier>, notification=w131:T13)  [unwired: 2 in, 2 out]
        n145 = Unbundle By Name(w131) -> ("Action"=w127:T12)
        n146 = Equal?(x=4Pi_Dual_DM_-_Mode_Scan_-_Scan_Actions."Quit" ("y"), y=w127) -> (x = y?=w129:bool)
        n147 = while {
          shift-right: [w148] -> _
          shift-left: w127 -> [w142]
          tunnel: w135 -> [w147]
          tunnel: w134 -> [w146]
          tunnel: w130 -> [w145]
          tunnel: w126 -> [w140]
          shift-right: [w138] -> _
          shift-left: u16 0 -> [w139]
          shift-right: [w136] -> _
          shift-left: 0.0 -> [w137]
          stop <- w149 stop-if-true
          n148 = Get Notifier Status(notifier=w145) -> (notifier out=w144:refnum<notifier>, current notification=w143:T13)  [unwired: 1 in, 3 out]
          n149 = case shown="\"Exit\", \"Quit\"" w142 {
            selector: w142 -> [_ _ _ _ _ _ _ _ w413]
            tunnel: [w152 w171 w207 w264 w307 w315 w380 w404 TRUE] -> w149
            tunnel: [4Pi_Dual_DM_-_Mode_Scan_-_Scan_Actions."Update Mode Amount" ("y") 4Pi_Dual_DM_-_Mode_Scan_-_Scan_Actions."Get Image" ("y") w203 4Pi_Dual_DM_-_Mode_Scan_-_Scan_Actions."Update Counter" ("y") w308 4Pi_Dual_DM_-_Mode_Scan_-_Scan_Actions."Apply Correction" ("y") 4Pi_Dual_DM_-_Mode_Scan_-_Scan_Actions."Exit" ("y") 4Pi_Dual_DM_-_Mode_Scan_-_Scan_Actions."Scan Mode" ("y") 4Pi_Dual_DM_-_Mode_Scan_-_Scan_Actions."Exit" ("y")] -> w148
            tunnel: w147 -> [_ w176 _ _ _ _ w383 _ w411]
            tunnel: w146 -> [_ w174 w210 _ _ _ _ _ _]
            tunnel: w144 -> [_ _ _ _ _ _ _ _ w412]
            tunnel: w143 -> [w155 w172 w209 w268 _ w318 _ _ _]
            tunnel: FALSE -> [w152 w171 w207 w264 w307 w315 w380 w404 _]
            tunnel: w140 -> [_ _ w205 w263 _ _ _ _ _]
            tunnel: w139 -> [w151 w170 w202 w262 w306 w314 w379 w403 w410]
            tunnel: [w151 w170 w201 w262 w306 w314 w379 w403 w410] -> w138
            tunnel: w137 -> [w150 w169 w196 w260 w305 w313 w378 w402 w409]
            tunnel: [w150 w169 w195 w260 w305 w313 w378 w402 w409] -> w136
            frame "Scan Mode" {
              w159 = 4Pi_Dual_DM_-_Standard_Action."Read" ("Action")
              n150 = Unbundle By Name(w155) -> ("DM Scan Settings.Number of Steps"=w153:u16, "DM Scan Settings.Step Size (nm)"=w154:dbl)
              n151 = call "4Pi Dual DM - Mirror Mode DUAL AE.vi"("Action"=w159) -> ("Mirror Modes Out"=w161:T26)  [unwired: 14 in]
              n152 = call "4Pi Dual DM - Active Mirror AE.vi"("Action"=w159) -> ("Active Mirror"=w160:i32)  [unwired: 14 in]
              n153 = Index Array(array=w161, index (col)=w160) -> (element=w158:cluster{"Mode":string, "Amplitude":dbl}[])  [unwired: 1 in]
              n154 = Initialize Array(0.0 ("element"), 0 ("dimension size")) -> (w162:dbl[])
              n155 = call "4Pi Dual DM - Mode Scan Data AE.vi"("Amplitude"=w162, "Action"=4Pi_Dual_DM_-_Standard_Action."Write", "Metric"=w162) -> ()  [unwired: 11 in, 2 out]
              n156 = Index Array(array=w158, index="Current Mode") -> (element=w167:cluster{"Mode":string, "Amplitude":dbl})
              n157 = Unbundle By Name(w167) -> ("Amplitude"=w168:dbl)
              n158 = call "4Pi Dual DM - Mode Scan Counter.vi"("Center Value"=w168, "Action"=4Pi_Dual_DM_-_Standard_Counter_Action."Initialize", "Mode"="Current Mode", "Number of Steps"=w153, "Step Size"=w154) -> ()  [unwired: 8 in, 3 out]
            }
            frame "Update Mode Amount" {
              n159 = flat-sequence {
                tunnel: w176 -> [w187]
                tunnel: [w187] -> w175
                tunnel: w175 -> [w190]
                tunnel: w174 -> [w194]
                tunnel: w172 -> [w193]
                frame #0 {
                  w183 = 4Pi_Dual_DM_-_Standard_Action."Read" ("Action")
                  n160 = call "4Pi Dual DM - Mirror Mode DUAL AE.vi"("Action"=w183) -> ("Mirror Modes Out"=w180:T26)  [unwired: 14 in]
                  n161 = call "4Pi Dual DM - Active Mirror AE.vi"("Action"=w183) -> ("Active Mirror"=w177:i32)  [unwired: 14 in]
                  n162 = Index Array(array=w180, index (col)=w177) -> (element=w182:cluster{"Mode":string, "Amplitude":dbl}[])  [unwired: 1 in]
                  n163 = call "4Pi Dual DM - Mode Scan Counter.vi"("Action"=4Pi_Dual_DM_-_Standard_Counter_Action."Get Count") -> ("Mode Amount"=w184:dbl, "Current Mode"=w185:i32)  [unwired: 12 in, 1 out]
                  n164 = Index Array(array=w182, index=w185) -> (element=w188:cluster{"Mode":string, "Amplitude":dbl})
                  n165 = Bundle By Name(cluster=w188, "Amplitude"=w184) -> (w189:cluster{"Mode":string, "Amplitude":dbl})
                  n166 = Replace Array Subset(array=w182, new element=w189, index=w185) -> (w178:cluster{"Mode":string, "Amplitude":dbl}[])
                  n167 = Replace Array Subset(array=w180, new element=w178, index (col)=w177) -> (w179:T26)  [unwired: 1 in]
                  n168 = call "4Pi Dual DM - Mirror Mode DUAL AE.vi"("Action"=4Pi_Dual_DM_-_Standard_Action."Write", "Mirror Modes In"=w179) -> ()  [unwired: 13 in, 1 out]
                }
                frame #1 {
                  n169 = Enqueue Element(queue=w190, element="Mirror Modes" ("name (unnamed)")) -> ()  [unwired: 2 in, 3 out]
                }
                frame #2 {
                  n170 = Unbundle By Name(w193) -> ("DM Scan Settings.Frame Delay"=w192:u32)
                  n171 = call "4Pi Dual DM - Confirm New Frame.vi"("Camera Notifier Name"=w194, "Wait No. (1)"=w192) -> ()  [unwired: 12 in, 2 out]
                }
              }
            }
            frame "Get Image" {
              n172 = Unbundle By Name(w209) -> ("Image Type"=w206:T4, "Image Ref"=w208:T1, "Blink Scan Settings.Blink Analysis Type"=w199:T9, "Blink Scan Settings.Blink Threshold"=w198:sgl, "Blink Scan Settings.Blink ROI Box Width"=w197:u8, "DM Scan Settings.Frame Accumulations"=w200:u16)
              n173 = case shown="1" w206 {
                tunnel: w210 -> [w216 w227 w252]
                tunnel: w208 -> [w215 w226 w250]
                tunnel: w200 -> [w213 w225 w259]
                tunnel: w205 -> [w214 w223 _]
                tunnel: [w212 w220 w234] -> w204
                tunnel: [4Pi_Dual_DM_-_Mode_Scan_-_Scan_Actions."Compute Metric" ("y") 4Pi_Dual_DM_-_Mode_Scan_-_Scan_Actions."Compute Metric" ("y") w253] -> w203
                tunnel: w202 -> [w217 w221 w233]
                tunnel: [w217 w221 w256] -> w201
                tunnel: w198 -> [_ _ w249]
                tunnel: w199 -> [_ _ w238]
                tunnel: w197 -> [_ _ w243]
                tunnel: w196 -> [w211 w219 w231]
                tunnel: [w211 w219 w232] -> w195
                frame 0, Default {
                  # "Full Image"
                  n174 = call "4Pi Dual DM - Get Image Full.vi"("Camera Notifier Name"=w216, "Image Ref"=w215, "Image Dst"=w214, "Frame Accums."=w213) -> ("Image Dst Out"=w212:T1)  [unwired: 11 in]
                }
                frame 1 {
                  # "ROI"
                  n175 = call "4Pi Dual DM - Get Image ROI.vi"("Camera Notifier Name"=w227, "Image Ref"=w226, "Frame Accums."=w225) -> ("Image Out"=w224:u16[][])  [unwired: 12 in]
                  n176 = call "IMAQ ArrayToImage"("Image Pixels (U16)"=w224, "Image"=w223) -> ("Image Out"=w220:T1)  [unwired: 8 in, 1 out]
                }
                frame 2 {
                  # "Blinks"
                  n177 = Increment(x=w233) -> (x+1=w257:u16)
                  n178 = Equal To 0?(x=w233) -> (x = 0?=w229:bool)
                  n179 = call "4Pi Dual DM - Confirm New Frame.vi"("Camera Notifier Name"=w252, "Wait No. (1)"=u32 1) -> ("Error Out"=w248:errorcluster)  [unwired: 12 in, 1 out]
                  n180 = Greater Or Equal?(x=w257, y=w259) -> (x >= y?=w236:bool)
                  n181 = call "SMS Candidate Selection.vi"("Image Ref (U16)"=w250, "Blink Sensitivity"=w249, "Error In"=w248) -> ("Image Ref (U16) - Dup"=w234:T1, "Cadidate Image Ref"=w247:T1, "Error Out"=w246:errorcluster)  [unwired: 10 in]
                  n182 = Select(t=u16 0 ("f"), s=w236, f=w257) -> (s? t:f=w256:u16)
                  n183 = call "IMAQ DLL - Non Zero Indices.vi"("IMAQ Ref"=w247, "Error In"=w246) -> ("Row Column Indices"=w245:i32[][], "Error Out"=w244:errorcluster)  [unwired: 10 in, 2 out]
                  n184 = call "SMS Candidate Selection - Locations to ROIs.vi"("Image Ref"=w234, "Row Column Indices"=w245, "Error"=w244, "Box Half Size"=w243) -> ("Image Ref (DUP)"=w241:T1, "Image ROIs"=w242:T27, "ROI Coordinates (Left, Top, Right, Bottom)"=w240:i32[][], "Error Out"=w239:errorcluster)  [unwired: 8 in]
                  n185 = call "SMS Candidate Selection - Pull Sub Regions.vi"("Image Ref"=w241, "ROI Coordinates"=w240, "Error"=w239) -> ("ROIs"=w237:u16[][][])  [unwired: 10 in, 2 out]
                  n186 = property on="AO Image Display" class="ImageControl"("ROI"=w242) -> ()  [unwired: 2 in, 2 out]
                  n187 = Select(t=0.0, s=w229, f=w231) -> (s? t:f=w228:dbl)
                  n188 = call "4Pi Dual DM - Fit Sum ROIs.vi"("Blink Analysis Type"=w238, "ROIs"=w237) -> ("Blink Metric"=w230:dbl)  [unwired: 13 in]
                  n189 = Add(x=w230, y=w228) -> (x+y=w232:dbl)
                  n190 = Select(t=4Pi_Dual_DM_-_Mode_Scan_-_Scan_Actions."Compute Metric" ("y"), s=w236, f=4Pi_Dual_DM_-_Mode_Scan_-_Scan_Actions."Get Image") -> (s? t:f=w253:T12)
                }
              }
              "AO Image Display" <- w204
            }
            frame "Compute Metric" {
              n191 = Unbundle By Name(w268) -> ("Image Type"=w261:T4, "Metric"=w267:T5, "Threshold Mean Limits.Upper Limit"=w266:dbl, "Threshold Mean Limits.Lower Limit"=w265:dbl)
              n192 = case shown="Default" w261 {
                tunnel: [w287 w304] -> w275
                tunnel: w267 -> [w285 _]
                tunnel: w266 -> [w284 _]
                tunnel: w265 -> [w283 _]
                tunnel: w263 -> [w282 _]
                tunnel: w260 -> [_ w304]
                frame Default {
                  n193 = call "IMAQ ImageToArray"("Image"=w282) -> ("Image Pixels (U16)"=w281:u16[][])  [unwired: 3 in, 4 out]
                  n194 = To Double Precision Float(number=w281) -> (double precision float=w286:dbl[][])
                  n195 = case shown="3" w285 {
                    tunnel: w286 -> [w290 w293 w298 w302]
                    tunnel: [w288 w292 w296 w299] -> w287
                    tunnel: w284 -> [_ _ w295 _]
                    tunnel: w283 -> [_ _ w294 _]
                    frame 0, Default {
                      # "Max Pixel Value"
                      n196 = Array Max & Min(array=w290) -> (max value=w289:dbl)  [unwired: 3 out]
                      n197 = To Double Precision Float(number=w289) -> (double precision float=w288:dbl)
                    }
                    frame 1 {
                      # "No Zero Mean"
                      n198 = call "4Pi Dual DM - No Zeros Mean.vi"("Image IN"=w293, "STDev Factor"=0.0) -> ("No Zero Mean"=w292:dbl)  [unwired: 13 in]
                    }
                    frame 2 {
                      # "Threshold Array Mean"
                      n199 = call "4Pi Dual DM - Threshold 2D Array.vi"("2D Array IN"=w298, "Upper Limit (Inclusive)"=w295, "Lower Limit (Inclusive)"=w294) -> ("Threshold Array Out"=w297:dbl[])  [unwired: 12 in]
                      n200 = call-poly <vilib>:"Mean.vi"("X"=w297) -> ("mean"=w296:dbl)  [unwired: 1 out]
                    }
                    frame 3 {
                      # "Mean"
                      n201 = Array Size(array=w302) -> (size(s)=w303:i32[])
                      n202 = Multiply Array Elements(1:w303) -> (0:w301:i32)
                      n203 = Reshape Array(w302, w301) -> (w300:dbl[])
                      n204 = call-poly <vilib>:"Mean.vi"("X"=w300) -> ("mean"=w299:dbl)  [unwired: 1 out]
                    }
                  }
                }
                frame 2 {
                }
              }
              n205 = call "4Pi Dual DM - Mode Scan Data AE.vi"("Action"=4Pi_Dual_DM_-_Standard_Action."Read") -> ("Amplitude Out"=w272:dbl[], "Metric Out"=w273:dbl[])  [unwired: 13 in]
              n206 = call "4Pi Dual DM - Mode Scan Counter.vi"("Action"=4Pi_Dual_DM_-_Standard_Counter_Action."Get Count") -> ("Mode Amount"=w274:dbl)  [unwired: 12 in, 2 out]
              n207 = Build Array (concatenate)(w273, w275) -> (w278:dbl[])
              n208 = Build Array (concatenate)(w272, w274) -> (w277:dbl[])
              n209 = call "4Pi Dual DM - Mode Scan Data AE.vi"("Amplitude"=w277, "Action"=4Pi_Dual_DM_-_Standard_Action."Write", "Metric"=w278) -> ()  [unwired: 11 in, 2 out]
              n210 = Bundle(w277, w278) -> (w279:cluster{dbl[], dbl[]})  [unwired: 1 in]
              n211 = Build Array(w279) -> (→"Metric":cluster{dbl[], dbl[]}[])
            }
            frame "Update Counter" {
              n212 = call "4Pi Dual DM - Mode Scan Counter.vi"("Action"=4Pi_Dual_DM_-_Standard_Counter_Action."Update Count") -> ("Scan Done?"=w311:bool)  [unwired: 12 in, 2 out]
              n213 = Select(t=4Pi_Dual_DM_-_Mode_Scan_-_Scan_Actions."Fit Data" ("y"), s=w311, f=4Pi_Dual_DM_-_Mode_Scan_-_Scan_Actions."Update Mode Amount" ("y")) -> (s? t:f=w308:T12)
            }
            frame "Fit Data" {
              n214 = Unbundle By Name(w318) -> ("Gaussian Initial Guesses"=w317:T2, "Fit Type"=w316:T6)
              n215 = call "4Pi Dual DM - Mode Scan Data AE.vi"("Action"=4Pi_Dual_DM_-_Standard_Action."Read") -> ("Amplitude Out"=w328:dbl[], "Metric Out"=w329:dbl[])  [unwired: 13 in]
              n216 = Bundle("Amplitude Out"=w328, "Metric Out"=w329) -> (w327:T28)  [unwired: 1 in]
              n217 = case shown="0, Default" w316 {
                tunnel: w328 -> [w333 w377]
                tunnel: w329 -> [w361 w376]
                tunnel: [w352 w373] -> w322
                tunnel: [w351 w374] -> w325
                tunnel: [w350 w375] -> w324
                tunnel: w317 -> [w348 _]
                frame 0, Default {
                  n218 = To Double Precision Float(number=w361) -> (double precision float=w360:dbl[])
                  n219 = Array Max & Min(array=w333) -> (max value=w339:dbl, min value=w338:dbl)  [unwired: 2 out]
                  n220 = Unbundle By Name(w348) -> ("Amplitude"=w347:dbl, "Center Position"=w346:dbl, "Width (Sigma)"=w345:dbl, "Offset"=w344:dbl, "User Guesses"=w331:bool)
                  n221 = Array Max & Min(array=w360) -> (max value=w341:dbl, max index (indices)=w334:i32, min value=w340:dbl)  [unwired: 1 out]
                  n222 = Subtract(x=w339, y=w338) -> (x-y=w337:dbl)
                  n223 = Divide(x=w337, y=2.0) -> (x/y=w335:dbl)
                  n224 = Bundle By Name(cluster=T23 {"initial amplitude"=nan, "initial center"=nan, "initial standard deviation"=nan, "offset"=nan} ("initial guess"), "initial amplitude"=w347, "initial center"=w346, "initial standard deviation"=w345, "offset"=w344) -> (w342:T23)
                  n225 = Index Array(array=w333, index=w334) -> (element=w332:dbl)
                  n226 = Bundle(w341, "Numeric"=w332, w335, w340) -> (w359:cluster{dbl, "Numeric":dbl, dbl, dbl})  [unwired: 1 in]
                  n227 = Select(t=w342, s=w331, f=w359) -> (s? t:f=w343:T29)
                  n228 = call <vilib>:"Gaussian Peak Fit.vi"("Y"=w360, "initial guess"=w343, "X"=w333, "parameter bounds"=T24 {"amp min"=0.0, "amp max"=100000.0, "center min"=-100.0, "center max"=100.0, "deviation min"=0.0, "deviation max"=1000.0, "offset min"=0.0, "offset max"=1000.0}) -> ("offset"=w355:dbl, "amplitude"=w357:dbl, "center"=w352:dbl, "standard deviation"=w356:dbl)  [unwired: 5 in, 3 out]
                  n229 = Build Array(w357, w352, w356, w355) -> (w354:dbl[])
                  n230 = call "4Pi Dual DM - 1D Gaussian.vi"("Parameters In"=w354, "Number of Points"=1000.0, "Max X Value"=w339, "Min X Value"=w338) -> ("X Values"=w351:dbl[], "Y Values"=w350:dbl[])  [unwired: 10 in]
                }
                frame 1 {
                  w371 = T30 2 items=["Least Square", "Least Absolute Residual", "Bisquare"] ("method")
                  # "LV often can't find this file. It should be located at C:\\Program Files\\National Instruments\\LabVIEW 2016\\examples\\Mathematics\\Fitting\\support"
                  n231 = To Double Precision Float(number=w376) -> (double precision float=w372:dbl[])
                  n232 = call <vilib>:"General Polynomial Fit.vi"("Y"=w372, "polynomial order"=2, "X"=w377, "method"=w371) -> ("Polynomial Coefficients"=w368:dbl[])  [unwired: 8 in, 3 out]
                  n233 = Array Max & Min(array=w377) -> (max value=w364:dbl, min value=w363:dbl)  [unwired: 2 out]
                  n234 = call "NI- Regression Equation String.vi"("coefficients"=w368, "precision"=3, "fit type"=T25."Polynomial") -> ("Formula"=w366:string)  [unwired: 8 in]
                  n235 = call <vilib>:"Eval y=f(x) Optimal Step.vi"("number of points"=u32 3000, "formula"=w366, "end"=w364, "start"=w363) -> ("Y Values"=w375:dbl[], "X Values"=w374:dbl[])  [unwired: 1 in, 2 out]
                  n236 = Array Max & Min(array=w375) -> (max index (indices)=w362:i32)  [unwired: 3 out]
                  n237 = Index Array(array=w374, index=w362) -> (element=w373:dbl)
                }
              }
              n238 = Bundle("X Values"=w325, "Y Values"=w324) -> (w323:cluster{"X Values":dbl[], "Y Values":dbl[]})  [unwired: 1 in]
              n239 = Build Array(w327, w323) -> (w326:cluster{"X Values":dbl[], "Y Values":dbl[]}[])
              n240 = property on="Metric" class="XYGraph (strict)"("Cursor.Cursor X"=w322, "Cursor.Cursor Y"=-10000.0 ("Cursor.Cursor Position:Cursor X"), "Cursor.Visible"=TRUE, "Value"=w326) -> ()  [unwired: 2 in, 2 out]
            }
            frame "Apply Correction" {
              n241 = flat-sequence {
                tunnel: w383 -> [w399]
                tunnel: [w399] -> w382
                tunnel: w382 -> [w400]
                frame #0 {
                  w392 = 4Pi_Dual_DM_-_Standard_Action."Read" ("Action")
                  n242 = property on="Metric" class="XYGraph (strict)"() -> ("Cursor.Cursor X"=w384:dbl)  [unwired: 2 in, 2 out]
                  n243 = call "4Pi Dual DM - Mirror Mode DUAL AE.vi"("Action"=w392) -> ("Mirror Modes Out"=w395:T26)  [unwired: 14 in]
                  n244 = call "4Pi Dual DM - Active Mirror AE.vi"("Action"=w392) -> ("Active Mirror"=w398:i32)  [unwired: 14 in]
                  n245 = Not A Number/Path/Refnum?(number/path/refnum=w384) -> (NaN/Path/Refnum?=w386:bool)
                  n246 = Index Array(array=w395, index (col)=w398) -> (element=w393:cluster{"Mode":string, "Amplitude":dbl}[])  [unwired: 1 in]
                  n247 = Select(t=0.0, s=w386, f=w384) -> (s? t:f=w387:dbl)
                  n248 = call "4Pi Dual DM - Mode Scan Counter.vi"("Action"=4Pi_Dual_DM_-_Standard_Counter_Action."Get Count") -> ("Current Mode"=w391:i32)  [unwired: 12 in, 2 out]
                  n249 = Index Array(array=w393, index=w391) -> (element=w389:cluster{"Mode":string, "Amplitude":dbl})
                  n250 = Bundle By Name(cluster=w389, "Amplitude"=w387) -> (w388:cluster{"Mode":string, "Amplitude":dbl})
                  n251 = Replace Array Subset(array=w393, new element=w388, index=w391) -> (w397:cluster{"Mode":string, "Amplitude":dbl}[])
                  n252 = Replace Array Subset(array=w395, new element=w397, index (col)=w398) -> (w396:T26)  [unwired: 1 in]
                  n253 = call "4Pi Dual DM - Mirror Mode DUAL AE.vi"("Action"=4Pi_Dual_DM_-_Standard_Action."Write", "Mirror Modes In"=w396) -> ()  [unwired: 13 in, 1 out]
                }
                frame #1 {
                  n254 = Enqueue Element(queue=w400, element="Mirror Modes" ("name (unnamed)")) -> ()  [unwired: 2 in, 3 out]
                }
              }
            }
            frame "Scan Next Mode" {
              n255 = call "4Pi Dual DM - Mode Scan Counter.vi"("Action"=4Pi_Dual_DM_-_Standard_Counter_Action."Get Count") -> ("Current Mode"=w407:i32)  [unwired: 12 in, 2 out]
              n256 = Increment(x=w407) -> (x+1=w408:i32)
              n257 = local write "Current Mode"(w408) -> ()
            }
            frame "Exit", "Quit" {
              n258 = case shown="\"Quit\"" w413 {
                tunnel: w412 -> [w434 _]
                tunnel: w411 -> [w435 _]
                frame "Quit" {
                  w432 = T14 {"Image Ref Index"=0, "Image Type"=0, "Fit Type"=0, "Metric"=1, "DM Scan Settings"={"Frame Delay"=1, "Frame Accumulations"=2, "Number of Steps"=8, "Step Size (nm)"=80.0}, "Threshold Mean Limits"={"Upper Limit"=10000.0, "Lower Limit"=0.0}, "Gaussian Initial Guesses"={"Amplitude"=2500.0, "Center Position"=0.0, "Width (Sigma)"=200.0, "Offset"=500.0, "User Guesses"=TRUE}, "Blink Scan Settings"={"Blink Analysis Type"=1, "Blink ROI Box Width"=0, "Blink Threshold"=0.0}}  # Last Used Scan Settings
                  n259 = Release Notifier(notifier=w434, force destroy? (F)=TRUE) -> (last notification=w433:T13)  [unwired: 1 in, 2 out]
                  n260 = Release Queue(queue=w435) -> ()  [unwired: 2 in, 3 out]
                  n261 = Unbundle By Name(w433) -> ("Image Type"=w431:T4, "Fit Type"=w429:T6, "Metric"=w428:T5, "DM Scan Settings"=w427:T3, "Threshold Mean Limits"=w426:T7, "Gaussian Initial Guesses"=w425:T2, "Blink Scan Settings"=w424:T8)
                  n262 = local read "Image Selection"() -> (w430:i32)
                  n263 = control-ref of="This VI"() -> (w423:refnum<vi>)
                  n264 = property class="VI"(reference=w423) -> ("Path"=w422:path)  [unwired: 1 in, 2 out]
                  n265 = Bundle By Name(cluster=w432, "Image Ref Index"=w430, "Image Type"=w431, "Fit Type"=w429, "Metric"=w428, "DM Scan Settings"=w427, "Threshold Mean Limits"=w426, "Gaussian Initial Guesses"=w425, "Blink Scan Settings"=w424) -> (w418:T14)
                  n266 = Strip Path(path=w422) -> (stripped path=w421:path)  [unwired: 1 out]
                  n267 = Strip Path(path=w421) -> (stripped path=w420:path)  [unwired: 1 out]
                  n268 = Build Path(base path=w420, name or relative path="4Pi Dual DM - Default Files\\Last Used Scan Settings.json") -> (appended path=w416:path)
                  n269 = Flatten To JSON(anything=w418) -> (JSON string=w417:string)  [unwired: 2 in, 1 out]
                  n270 = Write to Text File(file (use dialog)=w416, text=w417) -> ()  [unwired: 2 in, 3 out]
                }
                frame "Exit", Default {
                }
              }
            }
          }
        }
      }
      n271 = call "IMAQ Dispose"("Image"=w117) -> ()  [unwired: 5 in, 1 out]
    }
    frame Error {
      n272 = Release Notifier(notifier=w565) -> ()  [unwired: 2 in, 3 out]
      n273 = Release Notifier(notifier=w566) -> ()  [unwired: 2 in, 3 out]
      n274 = Release Queue(queue=w567) -> ()  [unwired: 2 in, 3 out]
      n275 = call "IMAQ Dispose"("Image"=w568) -> ()  [unwired: 5 in, 1 out]
    }
  }
